vi "DumpSendData.vi"(10 "Data":dbl[][](array[numeric]), 11 "DumpFileQueue":T1) -> ()   [LabVIEW 2025]
uses:
  DumpFileQueue.ctl
  DumpFileEvent.ctl
  DumpFileAction.ctl
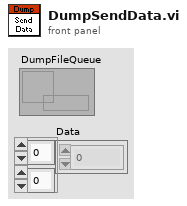
[diagram p1: front panel]
types:
  T1 = typedef "DumpFileQueue.ctl" = refnum<queue>
  T2 = typedef "DumpFileAction.ctl" = enum16{"StartNew", "StartAppend", "Data", "Close"}
  T3 = typedef "DumpFileEvent.ctl" = cluster{"Path":path, "DumpFileAction":T2, "Data":dbl[][]}
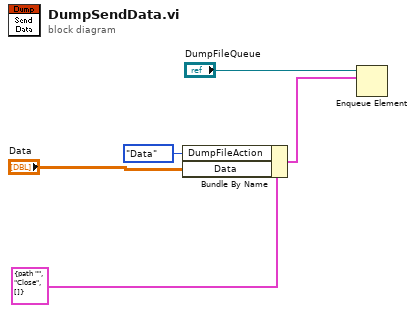
[diagram p0: block diagram]
diagram:
  n1 = Bundle By Name(cluster=T3 {"Path"=path "", "DumpFileAction"=enum."Close", "Data"=[]} ("element"), "DumpFileAction"=DumpFileAction."Data", "Data"="Data") -> (w3:T3)
  n2 = Enqueue Element(queue="DumpFileQueue", element=w3) -> ()  [unwired: 2 in, 3 out]
